vi "Region Sequence Anaysis.vi"(8 "Base Ex Info":T4, 9 "std":cluster{"CP std (%)":dbl, "P std (%)":dbl}={"CP std (%)"=0.02, "P std (%)"=0.02} {"P std (%)" format="%#_13g"; "CP std (%)" format="%#_13g"}, 11 "Relative Data Array":dbl[](array[numeric])) -> (0 "CP Analysis":T6, 1 "Assinged Signal Profile plus":T3, 2 "Assigned CP Profile plus":T1, 3 "Change Point Array":T7, 4 "CP Probability":dbl[][](array[numeric]), 5 "Assigned Time Profile plus":T2, 6 "Time Probability":dbl[][](array[numeric]))   [LabVIEW 2018]
uses:
  <vilib>/regexp/Match Regular Expression.xnode
  <vilib>/Analysis/NI_AALBase.lvlib
panel:
  out "CP ASCII_q":string[](array[string])
  out "Asciiq Sequence":string[](array[string])
  out "length":i32
  out "All ascii q Assigned":string
  out "S CP IDX End":i32[](array[numeric])
  out "S CP IDX Start":i32[](array[numeric])
  out "S S IDX":i32[](array[numeric])
  out "CP T IDX":i32[](array[numeric])
  out "CP CP IDX":i32[](array[numeric])
  out "T T IDX":i32[](array[numeric])
  out "CP S IDX":i32[](array[numeric])
  out "T S IDX":i32[](array[numeric])
  out "T CP IDX":i32[](array[numeric])
  out "Signal Time Sequence":string[](array[string])
  out "Signal Time length":i32[](array[numeric])
  out "Signal Q":dbl[](array[numeric])
  out "Signal Probability":dbl[](array[numeric])
  out "Signal Base length":i32[](array[numeric])
  out "Signal Sequence":string[](array[string])
  out "Assigned CP Profile":T5
  out "CP_Q value":dbl[](array[numeric])
  out "CP Probability":dbl[](array[numeric])
  out "CP Base":string[](array[string])
  out "CP assigned lvl":dbl[](array[numeric])
  out "CP Poiint Count":i32[](array[numeric])
  out "CP Region STD":dbl[](array[numeric])
  out "CP Relative Data Average":dbl[](array[numeric])
  out "B omit":string
  out "シグナル途中終了ではない":bool
  out "シグナル途中開始ではない":bool
  out "シグナル終了数":i32
  out "Signal END  IDX":i32[](array[numeric])
  out "シグナル開始数":i32
  out "転換点数":i32
  out "Signal Start IDX":i32[](array[numeric])
  out "Chang Point IDX":i32[](array[numeric])
  out "連続部位除去":string
  out "部分文字列":string
  out "部分文字列 2":string
  out "長さ":i32
  out "All P Assigned":string
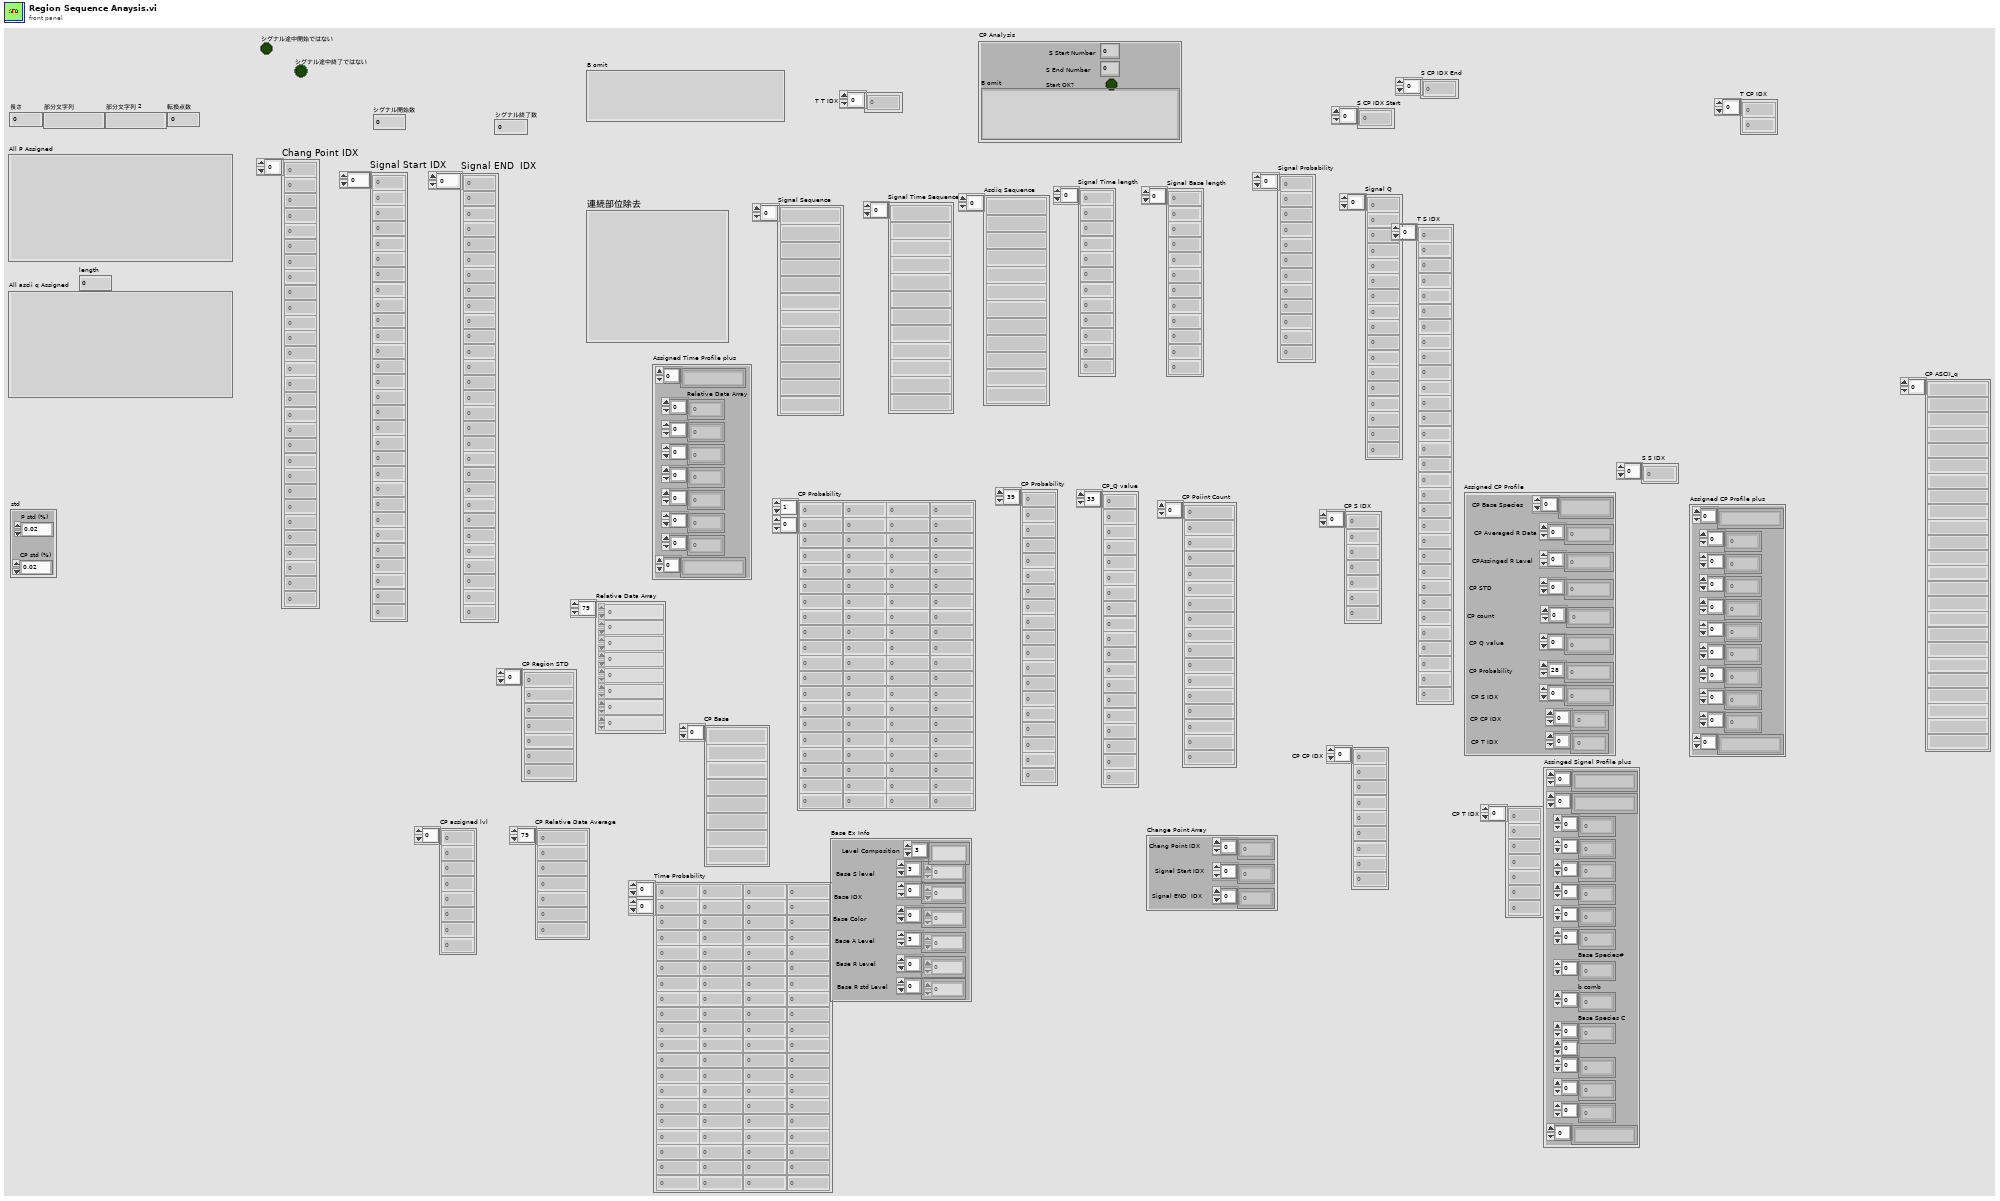
[diagram p1: front panel]
types:
  T1 = cluster{string[], dbl[], dbl[], dbl[], i32[], dbl[], dbl[], i32[], i32[], i32[], string[]}
  T2 = cluster{string[], "Relative Data Array":dbl[], dbl[], dbl[], dbl[], i32[], i32[], i32[], string[]}
  T3 = cluster{string[], string[], i32[], i32[], i32[], i32[], dbl[], dbl[], "Base Species#":i16[], "b comb":u32[], "Base Species C":i32[][], i32[], i32[], i32[], string[]}
  T4 = cluster{"Level Composition":string[], "Base S level":dbl[], "Base IDX":i32[], "Base Color":u32[], "Base A Level":dbl[], "Base R Level":dbl[], "Base R std Level":dbl[]}
  T5 = cluster{"CP Base Species":string[], "CP Averaged R Data":dbl[], "CPAssinged R Level":dbl[], "CP STD":dbl[], "CP count":i32[], "CP Q value":dbl[], "CP Probability":dbl[], "CP S IDX":i32[], "CP CP IDX":i32[], "CP T IDX":i32[]}
  T6 = cluster{"S Start Number":i32, "S End Number":i32, "Start OK?":bool, "End OK?":bool, "B omit":string}
  T7 = cluster{"Chang Point IDX":i32[], "Signal Start IDX":i32[], "Signal END  IDX":i32[]}
  T8 = cluster{i32[], dbl[], dbl[], string[], dbl[], string[]}
  T9 = cluster{"Level IDX":i32[], "Probability":dbl[], "Q value":dbl[], "Base Species":string[], "R level":dbl[]}
  T10 = cluster{string[], dbl[], dbl[], dbl[], i32[], dbl[], dbl[], i32[], i32[], i32[]}
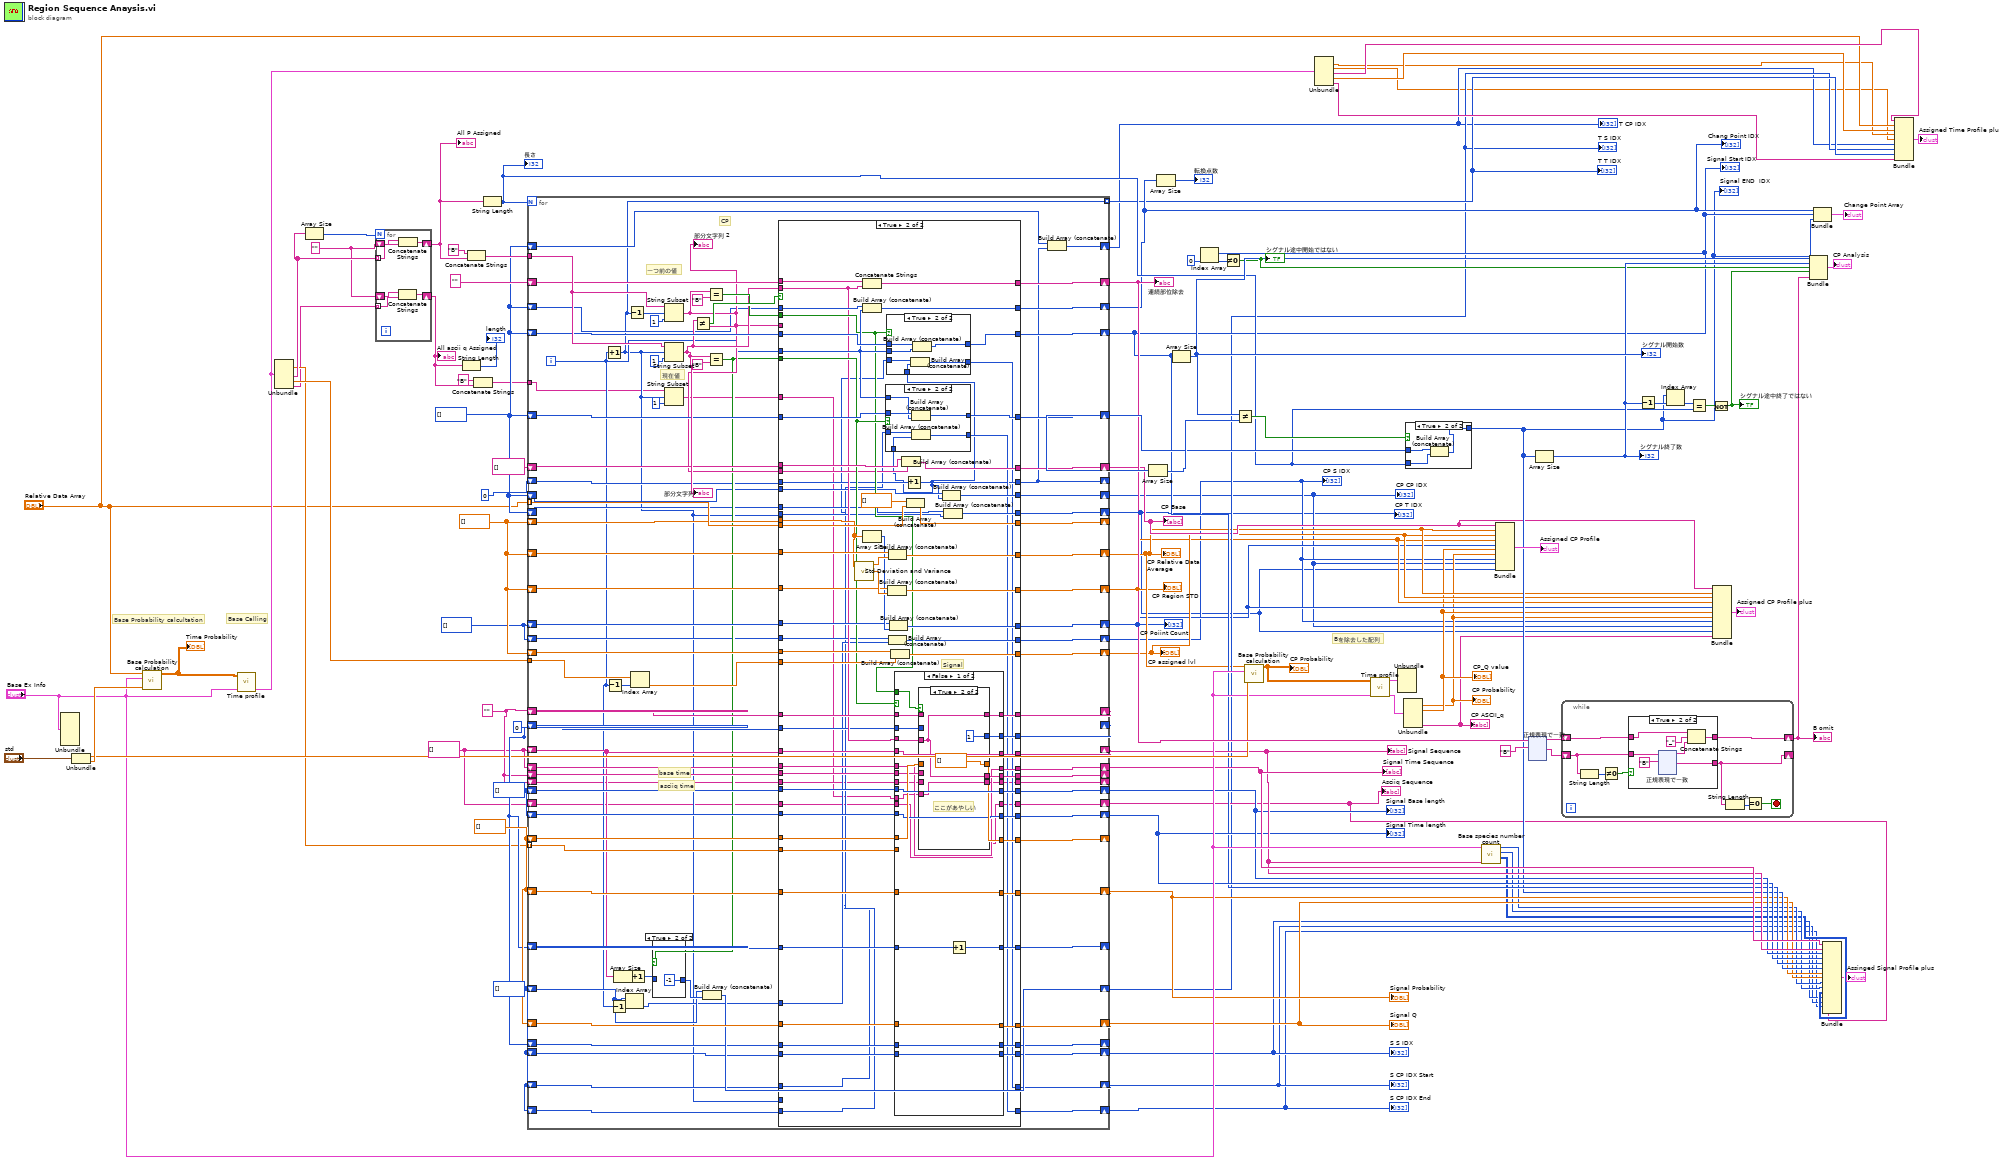
[diagram p0: block diagram]
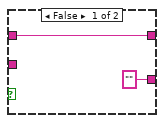
[diagram p2: hidden frame]
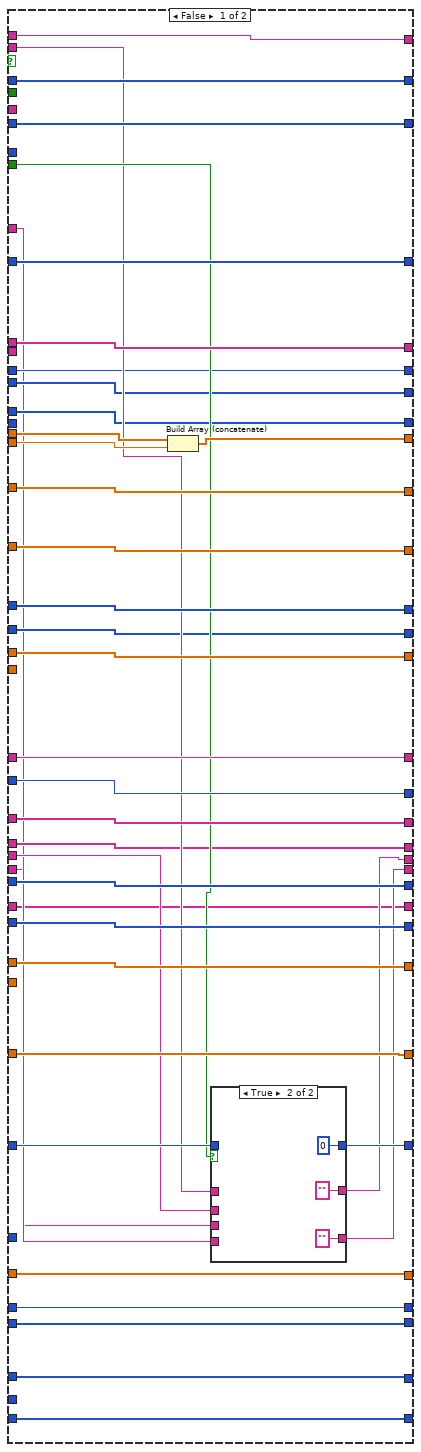
[diagram p5: hidden frame]
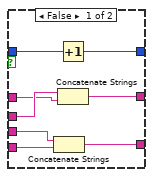
[diagram p6: hidden frame]
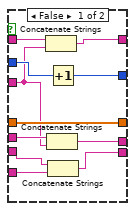
[diagram p7: hidden frame]
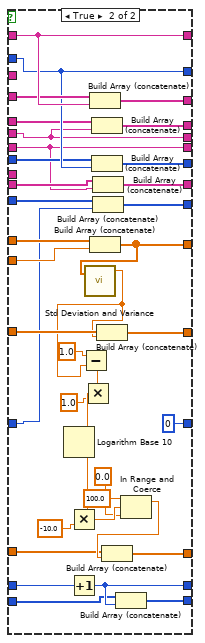
[diagram p8: hidden frame]
diagram:
  w57 = i32[] []
  w65 = dbl[] []
  w64 = i32[] []
  w58 = 0
  w41 = string[] []
  w42 = ""
  w61 = i32[] []
  w71 = dbl[] []
  w47 = ""
  w52 = i32[] []
  # "Base Probability calcultation"
  # "Base Calling"
  # "Bを除去した配列"
  n1 = Unbundle("Base Ex Info") -> ()  [unwired: 7 out]
  n2 = Unbundle("std") -> ("CP std (%)"=w55:dbl, "P std (%)"=w56:dbl)
  n3 = call "Base Probability calculation.vi"("std [%]"=w56, "Base Ex Info"="Base Ex Info", "Relative Array"="Relative Data Array") -> ("Time Probability"=w53:dbl[][])  [unwired: 8 in]
  "Time Probability" <- w53
  n4 = call "Time profile.vi"("Base Ex Info"="Base Ex Info", "Time Probability"=w53) -> ("Assigned Profile_plus"=w24:T8)  [unwired: 8 in, 1 out]
  n5 = Unbundle(w24) -> (w49:dbl[], w50:string[], w51:dbl[], w48:string[])  [unwired: 2 out]
  n6 = Array Size(array=w50) -> (size(s)=w89:i32)
  n7 = for {
    N: w89 -> [_]
    tunnel: w50 -> [w101] mode=indexing
    shift-right: [w100] -> w72
    shift-left: w47 -> [w99]
    tunnel: w48 -> [w97] mode=indexing
    shift-right: [w98] -> w44
    shift-left: w47 -> [w96]
    n8 = Concatenate Strings(w96, w97) -> (w98:string)
    n9 = Concatenate Strings(w99, w101) -> (w100:string)
  }
  "All P Assigned" <- w72
  "All ascii q Assigned" <- w44
  n10 = String Length(string=w44) -> (length=→"length":i32)
  n11 = Concatenate Strings("B" ("文字列"), w72) -> (w93:string)
  n12 = Concatenate Strings("B" ("string"), w44) -> (w45:string)
  n13 = String Length(string=w72) -> (length=w70:i32)
  "長さ" <- w70
  n14 = for {
    N: w70 -> [_]
    tunnel: w93 -> [w191]
    shift-right: [w188] -> w74
    shift-left: "" -> [w187]
    shift-right: [w186] -> w62
    shift-left: w52 -> [w138]
    shift-right: [w183] -> w36
    shift-left: w52 -> [w182]
    shift-right: [w178] -> w90
    shift-left: w52 -> [w179]
    tunnel: "Relative Data Array" -> [w176] mode=indexing
    shift-right: [w177] -> _
    shift-left: w71 -> [w175]
    shift-right: [w174] -> w11
    shift-left: w71 -> [w173]
    shift-right: [w172] -> w9
    shift-left: w71 -> [w171]
    shift-right: [w170] -> w8
    shift-left: w61 -> [w169]
    tunnel: w51 -> [w166]
    shift-right: [w168] -> w10
    shift-left: w71 -> [w167]
    shift-right: [w163] -> w12
    shift-left: string[] [] -> [w162]
    shift-right: [w159] -> _
    shift-left: w42 -> [w160]
    shift-right: [w158] -> w39
    shift-left: w41 -> [w135]
    shift-right: [w157] -> _
    shift-left: w58 -> [w156]
    shift-right: [w155] -> w38
    shift-left: w64 -> [w154]
    tunnel: w49 -> [w153] mode=indexing
    shift-right: [w152] -> _
    shift-left: w65 -> [w151]
    shift-right: [w150] -> w34
    shift-left: w65 -> [w149]
    shift-right: [w148] -> w33
    shift-left: w65 -> [w147]
    shift-right: [w146] -> _
    shift-left: w58 -> [w145]
    shift-right: [w144] -> w37
    shift-left: w64 -> [w143]
    shift-right: [w142] -> _
    shift-left: w42 -> [w141]
    shift-right: [w140] -> w40
    shift-left: w41 -> [w139]
    shift-right: [w136] -> w16
    shift-left: w52 -> [w137]
    shift-right: [w132] -> w17
    shift-left: w57 -> [w117]
    shift-right: [w130] -> w5
    shift-left: w61 -> [w129]
    tunnel: [w107] -> w18 mode=indexing
    shift-right: [w118] -> _
    shift-left: 0 ("y") -> [w128]
    shift-right: [w127] -> w4
    shift-left: w52 -> [w126]
    shift-right: [w125] -> w3
    shift-left: w52 -> [w124]
    shift-right: [w123] -> _
    shift-left: w58 -> [w122]
    shift-right: [w121] -> w29
    shift-left: w57 -> [w120]
    shift-right: [w112] -> w28
    shift-left: w57 -> [w113]
    shift-right: [w110] -> w27
    shift-left: w57 -> [w111]
    tunnel: w45 -> [w106]
    shift-right: [w108] -> _
    shift-left: w42 -> [w109]
    shift-right: [w102] -> w26
    shift-left: w41 -> [w103]
    i -> [w116]
    # "asciiq time"
    # "base time"
    # "CP"
    # "一つ前の値"
    # "現在値"
    n15 = Increment(x=w116) -> (x+1=w107:i32)
    n16 = Decrement(x=w116) -> (x-1=w164:i32)
    n17 = Decrement(x=w116) -> (x-1=w114:i32)
    n18 = Array Size(array=w135) -> (size(s)=w133:i32)
    n19 = Index Array(array=w117, index=w114) -> (element=w115:i32)
    n20 = Decrement(x=w107) -> (x-1=w192:i32)
    n21 = Increment(x=w133) -> (x+1=w119:i32)
    n22 = Index Array(array=w166, index=w164) -> (element=w165:dbl)
    n23 = String Subset(string=w191, offset (0)=w192, length (rest)=1 ("長さ（残り）")) -> (substring=w161:string)
    "部分文字列 2" <- w161
    n24 = String Subset(string=w191, offset (0)=w107, length (rest)=1 ("長さ（残り）")) -> (substring=w181:string)
    "部分文字列" <- w181
    n25 = String Subset(string=w106, offset (0)=w107, length (rest)=1 ("length (rest)")) -> (substring=w104:string)
    n26 = Not Equal?(x=w181, y=w161) -> (x != y?=w189:bool)
    n27 = Equal?(x=w161, y="B") -> (x = y?=w184:bool)
    n28 = Equal?(x=w181, y="B") -> (x = y?=w134:bool)
    n29 = case shown="True" w134 {
      tunnel: w119 -> [w194 _]
      tunnel: [w194 -1] -> w131
      frame False {
      }
      frame True {
      }
    }
    n30 = Build Array (concatenate)(w117, w131) -> (w132:i32[])
    n31 = case shown="True" w189 {
      tunnel: [w234 w322] -> w188
      tunnel: w187 -> [w234 w321]
      tunnel: w181 -> [w209 w289]
      tunnel: w116 -> [_ w314]
      tunnel: [w233 w319] -> w186
      tunnel: w138 -> [w233 w320]
      tunnel: w184 -> [_ w292]
      tunnel: [w232 w318] -> w183
      tunnel: w182 -> [w232 w317]
      tunnel: w134 -> [w212 w295]
      tunnel: w179 -> [w231 w316]
      tunnel: [w231 w315] -> w178
      tunnel: [w227 w313] -> w177
      tunnel: w176 -> [w229 w311]
      tunnel: w175 -> [w228 w304]
      tunnel: [w230 w310] -> w174
      tunnel: w173 -> [w230 w309]
      tunnel: [w226 w306] -> w172
      tunnel: w171 -> [w226 w305]
      tunnel: [w225 w302] -> w170
      tunnel: w169 -> [w225 w301]
      tunnel: w165 -> [_ w300]
      tunnel: [w224 w299] -> w168
      tunnel: w167 -> [w224 w298]
      tunnel: w161 -> [_ w291]
      tunnel: [w223 w296] -> w163
      tunnel: w162 -> [w223 w297]
      tunnel: w161 -> [_ _]
      tunnel: w160 -> [w222 w294]
      tunnel: [w222 w293] -> w159
      tunnel: [w221 w288] -> w158
      tunnel: w135 -> [w221 w290]
      tunnel: [w220 w287] -> w157
      tunnel: w156 -> [w220 w286]
      tunnel: [w219 w285] -> w155
      tunnel: w154 -> [w219 w284]
      tunnel: w153 -> [_ w283]
      tunnel: [w218 w282] -> w152
      tunnel: w151 -> [w218 w281]
      tunnel: [w217 w280] -> w150
      tunnel: w149 -> [w217 w279]
      tunnel: [w216 w278] -> w148
      tunnel: w147 -> [w216 w277]
      tunnel: [w213 w276] -> w146
      tunnel: w145 -> [w214 w275]
      tunnel: [w215 w274] -> w144
      tunnel: w143 -> [w215 w273]
      tunnel: [w210 w272] -> w142
      tunnel: w141 -> [w211 w271]
      tunnel: [w208 w270] -> w140
      tunnel: w139 -> [w208 w269]
      tunnel: w115 -> [_ w268]
      tunnel: [w207 w267] -> w130
      tunnel: w129 -> [w207 w266]
      tunnel: [w206 w253] -> w118
      tunnel: w128 -> [w206 w256]
      tunnel: [w205 w265] -> w127
      tunnel: w126 -> [w205 w264]
      tunnel: w107 -> [_ w263]
      tunnel: [w204 w262] -> w125
      tunnel: w124 -> [w204 w261]
      tunnel: [w203 w260] -> w123
      tunnel: w122 -> [w203 w259]
      tunnel: [w202 w258] -> w121
      tunnel: w120 -> [w202 w257]
      tunnel: w113 -> [w201 w251]
      tunnel: [w201 w252] -> w112
      tunnel: w111 -> [w200 w254]
      tunnel: [w200 w255] -> w110
      tunnel: w107 -> [_ _]
      tunnel: w109 -> [w198 w250]
      tunnel: [w197 w249] -> w108
      tunnel: w104 -> [w199 w246]
      tunnel: w103 -> [w196 w248]
      tunnel: [w196 w247] -> w102
      frame False {
        n32 = Build Array (concatenate)(w228, w229) -> (w227:dbl[])
        n33 = case shown="True" w212 {
          tunnel: w214 -> [w242 _]
          tunnel: [w241 0] -> w213
          tunnel: w211 -> [w240 _]
          tunnel: [w239 ""] -> w210
          tunnel: w209 -> [w238 _]
          tunnel: w199 -> [w237 _]
          tunnel: w198 -> [w236 _]
          tunnel: [w235 ""] -> w197
          frame False {
            n34 = Concatenate Strings(w236, w237) -> (w235:string)
            n35 = Increment(x=w242) -> (x+1=w241:i32)
            n36 = Concatenate Strings(w240, w238) -> (w239:string)
          }
          frame True {
          }
        }
      }
      frame True {
        # "Signal"
        n37 = call <vilib>:"Std Deviation and Variance.vi"("X"=w304) -> ("mean"=w308:dbl, "standard deviation"=w307:dbl)  [unwired: 1 in, 1 out]
        n38 = Concatenate Strings(w321, w289) -> (w322:string)
        n39 = Build Array (concatenate)(w320, w314) -> (w319:i32[])
        n40 = Array Size(array=w304) -> (size(s)=w303:i32)
        n41 = Build Array (concatenate)(w305, w307) -> (w306:dbl[])
        n42 = Build Array (concatenate)(w309, w308) -> (w310:dbl[])
        n43 = Build Array (concatenate)(w266, w268) -> (w267:i32[])
        n44 = Build Array (concatenate)(w301, w303) -> (w302:i32[])
        n45 = Build Array (concatenate)(w298, w300) -> (w299:dbl[])
        n46 = case shown="False" w295 {
          tunnel: w294 -> [w346 w399]
          tunnel: [w345 w399] -> w293
          tunnel: w292 -> [w344 _]
          tunnel: w289 -> [w343 _]
          tunnel: [w342 w398] -> w288
          tunnel: w290 -> [w342 w397]
          tunnel: [w341 w396] -> w287
          tunnel: w286 -> [w340 w396]
          tunnel: [w339 w395] -> w285
          tunnel: w284 -> [w339 w394]
          tunnel: w283 -> [_ w393]
          tunnel: [w337 w391] -> w282
          tunnel: w281 -> [w338 w392]
          tunnel: [w336 w390] -> w280
          tunnel: w279 -> [w336 w389]
          tunnel: [w335 w377] -> w278
          tunnel: w277 -> [w335 w376]
          tunnel: [w334 0] -> w276
          tunnel: w275 -> [w333 w375]
          tunnel: [w332 w374] -> w274
          tunnel: w273 -> [w332 w373]
          tunnel: [w331 w369] -> w272
          tunnel: w271 -> [w330 w369]
          tunnel: [w329 w371] -> w270
          tunnel: w269 -> [w329 w370]
          tunnel: [w328 w367] -> w260
          tunnel: w259 -> [w328 w368]
          tunnel: [w327 w366] -> w258
          tunnel: w257 -> [w327 w365]
          tunnel: w250 -> [w326 w362]
          tunnel: [w325 w362] -> w249
          tunnel: w248 -> [w324 w364]
          tunnel: [w324 w363] -> w247
          tunnel: w246 -> [w323 _]
          frame False {
            n47 = case shown="True" w344 {
              tunnel: w346 -> [w357 _]
              tunnel: [w356 w359] -> w345
              tunnel: w343 -> [w350 w359]
              tunnel: [w355 1] -> w341
              tunnel: w340 -> [w354 _]
              tunnel: w338 -> [w353 _]
              tunnel: [w353 dbl[] []] -> w337
              tunnel: [w352 w359] -> w331
              tunnel: w330 -> [w351 _]
              tunnel: w326 -> [w349 _]
              tunnel: [w348 w358] -> w325
              tunnel: w323 -> [w347 w358]
              frame False {
                n48 = Concatenate Strings(w357, w350) -> (w356:string)
                n49 = Concatenate Strings(w351, w350) -> (w352:string)
                n50 = Increment(x=w354) -> (x+1=w355:i32)
                n51 = Concatenate Strings(w349, w347) -> (w348:string)
              }
              frame True {
                # "ここがあやしい"
              }
            }
            n52 = Increment(x=w333) -> (x+1=w334:i32)
          }
          frame True {
            n53 = Increment(x=w368) -> (x+1=w367:i32)
            n54 = Build Array (concatenate)(w397, w399) -> (w398:string[])
            n55 = Build Array (concatenate)(w392, w393) -> (w391:dbl[])
            n56 = call <vilib>:"Std Deviation and Variance.vi"("X"=w391) -> ("mean"=w379:dbl)  [unwired: 1 in, 2 out]
            n57 = Subtract(x=1.0, y=w379) -> (x-y=w387:dbl)
            n58 = Multiply(x=w387, y=1.0) -> (x*y=w386:dbl)
            n59 = Logarithm Base 10(1:w386) -> (0:w388:dbl)
            n60 = Multiply(x=w388, y=-10.0) -> (x*y=w385:dbl)
            n61 = Build Array (concatenate)(w370, w369) -> (w371:string[])
            n62 = Build Array (concatenate)(w394, w396) -> (w395:i32[])
            n63 = Build Array (concatenate)(w364, w362) -> (w363:string[])
            n64 = Build Array (concatenate)(w373, w375) -> (w374:i32[])
            n65 = Build Array (concatenate)(w389, w379) -> (w390:dbl[])
            n66 = Build Array (concatenate)(w365, w367) -> (w366:i32[])
            n67 = In Range and Coerce(upper limit=100.0 ("上限"), x=w385, lower limit=0.0 ("下限")) -> (coerced(x)=w378:dbl)  [unwired: 1 out]
            n68 = Build Array (concatenate)(w376, w378) -> (w377:dbl[])
          }
        }
        n69 = Build Array (concatenate)(w297, w291) -> (w296:string[])
        n70 = Increment(x=w256) -> (x+1=w253:i32)
        n71 = case shown="True" w295 {
          tunnel: [w401 w407] -> w315
          tunnel: w316 -> [w401 w406]
          tunnel: w314 -> [_ w405]
          tunnel: [w400 w404] -> w255
          tunnel: w254 -> [w400 w403]
          tunnel: w253 -> [_ w402]
          frame False {
          }
          frame True {
            n72 = Build Array (concatenate)(w406, w405) -> (w407:i32[])
            n73 = Build Array (concatenate)(w403, w402) -> (w404:i32[])
          }
        }
        n74 = case shown="True" w292 {
          tunnel: [w409 w415] -> w318
          tunnel: w317 -> [w409 w414]
          tunnel: w314 -> [_ w413]
          tunnel: [w408 w412] -> w252
          tunnel: w251 -> [w408 w411]
          tunnel: w253 -> [_ w410]
          frame False {
          }
          frame True {
            n75 = Build Array (concatenate)(w411, w410) -> (w412:i32[])
            n76 = Build Array (concatenate)(w414, w413) -> (w415:i32[])
          }
        }
        n77 = Build Array (concatenate)(dbl[] [], w311) -> (w313:dbl[])
        n78 = Build Array (concatenate)(w264, w253) -> (w265:i32[])
        n79 = Build Array (concatenate)(w261, w263) -> (w262:i32[])
      }
    }
    n80 = Build Array (concatenate)(w137, w118) -> (w136:i32[])
  }
  "連続部位除去" <- w74
  "Chang Point IDX" <- w62
  "Signal Start IDX" <- w36
  "CP Relative Data Average" <- w11
  "CP Region STD" <- w9
  "CP Poiint Count" <- w8
  "CP assigned lvl" <- w10
  "CP Base" <- w12
  "Signal Sequence" <- w39
  "Signal Base length" <- w38
  "Signal Probability" <- w34
  "Signal Q" <- w33
  "Signal Time length" <- w37
  "Signal Time Sequence" <- w40
  "T CP IDX" <- w16
  "T S IDX" <- w17
  "CP S IDX" <- w5
  "T T IDX" <- w18
  "CP CP IDX" <- w4
  "CP T IDX" <- w3
  "S S IDX" <- w29
  "S CP IDX Start" <- w28
  "S CP IDX End" <- w27
  "Asciiq Sequence" <- w26
  n81 = Array Size(array=w90) -> (size(s)=w92:i32)
  n82 = Array Size(array=w62) -> (size(s)=→"転換点数":i32)
  n83 = Array Size(array=w36) -> (size(s)=w88:i32)
  "シグナル開始数" <- w88
  n84 = Index Array(array=w36, index=0 ("指標")) -> (element=w85:i32)
  n85 = Not Equal To 0?(x=w85) -> (x != 0?=w81:bool)
  "シグナル途中開始ではない" <- w81
  n86 = Not Equal?(x=w88, y=w92) -> (x != y?=w91:bool)
  n87 = call "Base Probability calculation.vi"("std [%]"=w55, "Base Ex Info"="Base Ex Info", "Relative Array"=w11) -> ("Time Probability"=w69:dbl[][])  [unwired: 8 in]
  "CP Probability" <- w69
  n88 = Unbundle(w24) -> (w20:dbl[], w15:dbl[], w23:string[], w21:dbl[], w19:string[])  [unwired: 1 out]
  n89 = call "Time profile.vi"("Base Ex Info"="Base Ex Info", "Time Probability"=w69) -> ("Assigned Profile_plus"=w13:T8, "Assigned Profile"=w68:T9)  [unwired: 8 in]
  n90 = Unbundle(w68) -> ()  [unwired: 5 out]
  n91 = Unbundle(w13) -> (w6:dbl[], w7:dbl[], w2:string[])  [unwired: 3 out]
  "CP Probability" <- w6
  "CP_Q value" <- w7
  "CP ASCII_q" <- w2
  n92 = case shown="True" w91 {
    tunnel: w90 -> [w416 w418]
    tunnel: [w416 w419] -> w35
    tunnel: w70 -> [_ w417]
    frame False {
    }
    frame True {
      n93 = Build Array (concatenate)(w418, w417) -> (w419:i32[])
    }
  }
  "Signal END  IDX" <- w35
  n94 = call "Base species number count.vi"("Signal Sequence"=w39, "Base Ex Info"="Base Ex Info") -> ("Base Species C"=w30:i32[][], "b comb"=w31:u32[], "Base Species#"=w32:i16[])  [unwired: 6 in, 1 out]
  n95 = Bundle(w12, w11, w10, w9, w8, w7, w6, w5, w4, w3) -> (→"Assigned CP Profile":T10)  [unwired: 1 in]
  n96 = xnode "正規表現で一致"("入力文字列"=w74, "正規表現"="B") -> ("一致の前"=w76:string, "一致の後"=w75:string)  [unwired: 4 in, 3 out]
  n97 = Array Size(array=w35) -> (size(s)=w84:i32)
  "シグナル終了数" <- w84
  n98 = while {
    shift-right: [w423] -> w63
    shift-left: w76 -> [w425]
    shift-right: [w422] -> _
    shift-left: w75 -> [w424]
    stop <- w420 stop-if-true
    n99 = String Length(string=w424) -> (length=w427:i32)
    n100 = Not Equal To 0?(x=w427) -> (x != 0?=w426:bool)
    n101 = case shown="True" w426 {
      tunnel: w425 -> [w429 w434]
      tunnel: w424 -> [_ w435]
      tunnel: ["" ("一致の後") w431] -> w422
      tunnel: [w429 w430] -> w423
      frame False {
      }
      frame True {
        n102 = xnode "正規表現で一致"("入力文字列"=w435, "正規表現"="B") -> ("一致の前"=w432:string, "一致の後"=w431:string)  [unwired: 4 in, 3 out]
        n103 = Concatenate Strings(w434, "_" ("文字列"), w432) -> (w430:string)
      }
    }
    n104 = String Length(string=w422) -> (length=w421:i32)
    n105 = Equal To 0?(x=w421) -> (x = 0?=w420:bool)
  }
  "B omit" <- w63
  n106 = Decrement(x=w84) -> (x-1=w83:i32)
  n107 = Index Array(array=w35, index=w83) -> (element=w82:i32)
  n108 = Equal?(x=w82, y=w70) -> (x = y?=w80:bool)
  n109 = Not(x=w80) -> (.not. x?=w78:bool)
  "シグナル途中終了ではない" <- w78
  n110 = Bundle(w12, w11, w10, w9, w8, w7, w6, w5, w4, w3, w2) -> (→"Assigned CP Profile plus":T1)  [unwired: 1 in]
  n111 = Bundle(w88, w84, w81, w78, "一致の前"=w63) -> (→"CP Analysis":cluster{i32, i32, bool, bool, "一致の前":string})  [unwired: 1 in]
  n112 = Bundle(w62, w36, w35) -> (→"Change Point Array":cluster{i32[], i32[], i32[]})  [unwired: 1 in]
  n113 = Bundle(w40, w39, w38, w37, w36, w35, w34, w33, "Base Species#"=w32, "b comb"=w31, "Base Species C"=w30, w29, w28, w27, w26) -> (→"Assinged Signal Profile plus":T3)  [unwired: 1 in]
  n114 = Bundle(w23, "Relative Data Array"="Relative Data Array", w21, w20, w15, w16, w17, w18, w19) -> (→"Assigned Time Profile plus":T2)  [unwired: 1 in]
